vi "calculate Search Range.vi"(8 "Search Width":dbl, 9 "Fundametal Freq":dbl) -> (2 "배열":cluster{"Start":dbl, "End":dbl}[](array[cluster]))   [LabVIEW 2023, in "Instrument Manager.lvclass"]
uses:
  Instrument Manager.lvclass
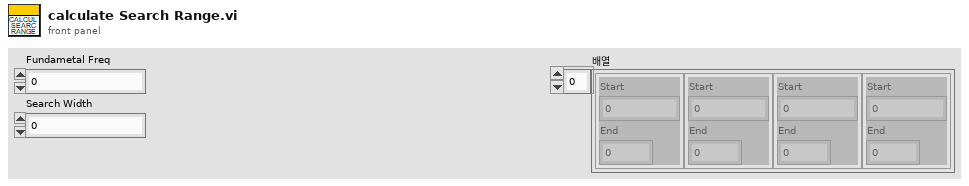
[diagram p1: front panel]
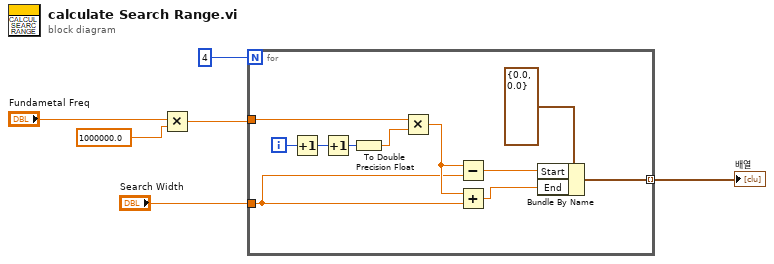
[diagram p0: block diagram]
diagram:
  n1 = Multiply(x="Fundametal Freq", y=1000000.0) -> (x*y=w2:dbl)
  n2 = for {
    N: 4 -> [_]
    tunnel: w2 -> [w17]
    tunnel: "Search Width" -> [w11]
    tunnel: [w7] -> w4 mode=indexing
    i -> [w16]
    n3 = Increment(x=w16) -> (x+1=w15:i32)
    n4 = Increment(x=w15) -> (x+1=w14:i32)
    n5 = To Double Precision Float(number=w14) -> (double precision float=w13:dbl)
    n6 = Multiply(x=w17, y=w13) -> (x*y=w12:dbl)
    n7 = Subtract(x=w12, y=w11) -> (x-y=w10:dbl)
    n8 = Add(x=w12, y=w11) -> (x+y=w9:dbl)
    n9 = Bundle By Name(cluster=cluster{"Start":dbl, "End":dbl} {"Start"=0.0, "End"=0.0} ("입력 클러스터"), "Start"=w10, "End"=w9) -> (w7:cluster{"Start":dbl, "End":dbl})
  }
  "배열" <- w4
